vi "NR set Center Channel.vi"(8 "error in (no error)":errorcluster caption="에러 입력(에러 없음)", 10 "Center Channel Number":u32, 11 "Instrument Manager 입력":refnum<class "Instrument Manager.lvclass">) -> (0 "error out":errorcluster caption="에러 출력", 3 "Instrument Manager 출력":refnum<class "Instrument Manager.lvclass">)   [LabVIEW 2023, in "Instrument Manager.lvclass"]
uses:
  Instrument Manager.lvclass
  Module/ANRITSU Call Box/Type Definition/NR Center Channel Arguments.ctl
  Module/ANRITSU Call Box/Type Definition/Uplink Downlink Enum.ctl
  Instrument Manager.lvclass/Instrument Manager.ctl
  Module/ANRITSU Call Box/Interface Class/Anritsu Call Box.lvclass
  Module/ANRITSU Call Box/ANRITSU Call Box.lvlib
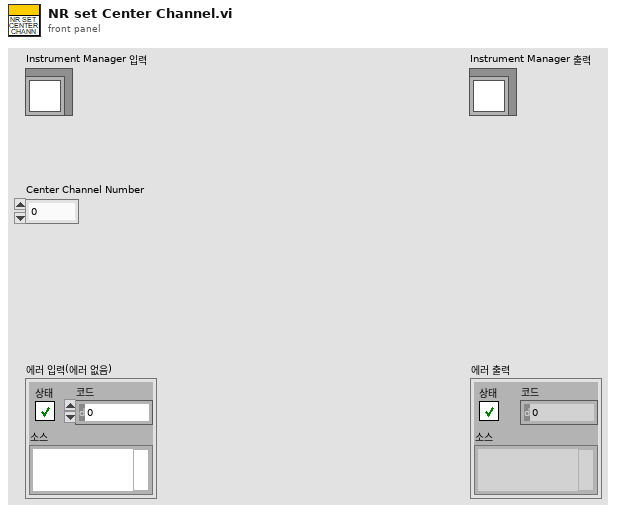
[diagram p1: front panel]
types:
  T1 = typedef "ANRITSU Call Box.lvlib/Uplink Downlink Enum.ctl" = enum16{"Uplink", "Downlink"}
  T2 = typedef "ANRITSU Call Box.lvlib/NR Center Channel Arguments.ctl" = cluster{"Center Channel Number":u32, "Selected CC":enum16{"PCC", "SCC", "FR2_PCC", "FR2_SCC"}, "SCC or FR2_SCC Index":u32}
  T3 = cluster{"Anritsu Call Box":refnum<class "Anritsu Call Box.lvclass">, "Spectrum Analyzer":refnum<class "Interface_Spectrum.lvclass">, "RF Switch Box":refnum<class "RF Filter Box.lvclass">, "Turn Table":refnum<class "Interface - Turn Table.lvclass">, "Mast":refnum<class "Interface - Mast.lvclass">, "3D Controller":refnum<class "Interface_3D Controller.lvclass">}
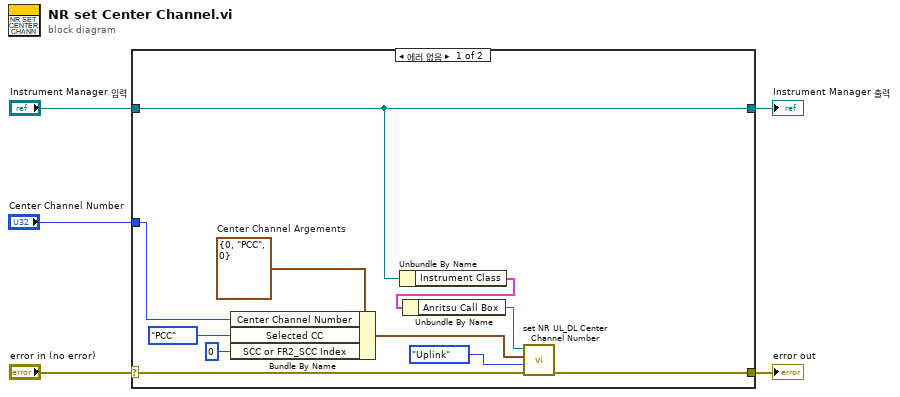
[diagram p0: block diagram]
diagram:
  n1 = case shown="에러 없음" "error in (no error)" {
    selector: "error in (no error)" -> [w12 w18]
    tunnel: [w6 w18] -> w4
    tunnel: [w11 w17] -> w2
    tunnel: "Instrument Manager 입력" -> [w11 w17]
    tunnel: "Center Channel Number" -> [w15 _]
    frame No Error {
      w16 = T2 {"Center Channel Number"=0, "Selected CC"=enum."PCC", "SCC or FR2_SCC Index"=0}  # Center Channel Argements
      n2 = Bundle By Name(cluster=w16, "Center Channel Number"=w15, "Selected CC"=enum16{"PCC", "SCC", "FR2_PCC", "FR2_SCC"}."PCC", "SCC or FR2_SCC Index"=u32 0) -> (w9:T2)
      n3 = Unbundle By Name(w11) -> ("Instrument Class"=w10:T3)
      n4 = Unbundle By Name(w10) -> ("Anritsu Call Box"=w7:refnum<class "Anritsu Call Box.lvclass">)
      n5 = call-dynamic "set NR UL_DL Center Channel Number.vi"("error in (no error)"=w12, "Direction"=Uplink_Downlink_Enum."Uplink", "Center Channel Argements"=w9, "Anritsu Call Box in"=w7) -> ("error out"=w6:errorcluster)  [unwired: 6 in, 1 out]
    }
    frame Error {
    }
  }
  "error out" <- w4
  "Instrument Manager 출력" <- w2
